vi "[ex ce] Eval y=f(x1,x2).vi"() -> ()   [LabVIEW 2021]
doc: "CE-Math example.\n\n::: CalcExpress Toolkit :::\nCopyright (c) 2000-2026 Konstantin Shifershteyn. All rights reserved."
uses:
  ce exmpl - 2D difference info.ctl
  <vilib>/gmath/NI_Gmath.lvlib
panel:
  out "max relative difference":T1 {"relative difference, %" format="%#.6g"; "absolute difference" format="%#.6g"}
  out "max absolute difference":T1 {"relative difference, %" format="%#.6g"; "absolute difference" format="%#.6g"}
  out "speed ratio":dbl format="%.3f"
  out "GM ticks":u32 caption="ms"
  out "CE ticks":u32 caption="ms"
  out "CE Graph":dbl[][](graph) caption="CalcExpress"
  in  "number of grid points for both variables":u32=100 min=10 max=500
  in  "parameters":cluster{"name":string, "value":dbl}[](array[cluster])=[{"name"="a", "value"=4.0}, {"name"="b", "value"=2.0}] {"value" format="%.2f"}
  in  "formula info":T2={"formula"="a*sinc(x1)-cos(b*x2+pi(1/2))", "variable 1"="x1", "variable 2"="x2"}
  in  "End":cluster{"x1":dbl, "x2":dbl}={"x1"=3.0, "x2"=3.0} {"x2" format="%.2f"; "x1" format="%.2f"}
  in  "Start":cluster{"x1":dbl, "x2":dbl}={"x1"=-3.0, "x2"=-3.0} {"x2" format="%.2f"; "x1" format="%.2f"}
  out "GM Graph":dbl[][](graph) caption="G Math"
  # "NOTE    CalcExpress uses (^) operator to perform bitwise-XOR operation but not power operation.\nYou have to use pow(x,y) function to compute the value of x raised to the y power in CalcExpress."
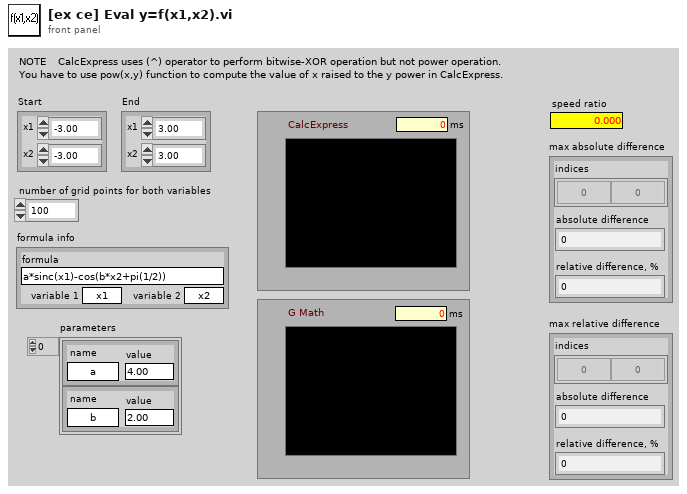
[diagram p1: front panel]
types:
  T1 = typedef "ce exmpl - 2D difference info.ctl" = cluster{"indices":i32[], "absolute difference":dbl, "relative difference, %":dbl}
  T2 = cluster{"formula":string, "variable 1":string, "variable 2":string}
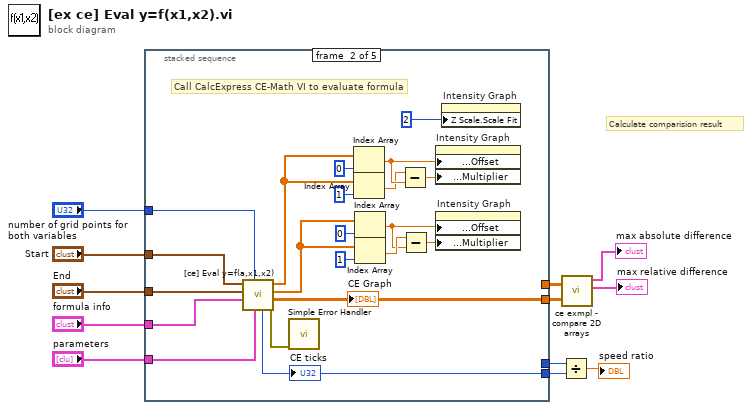
[diagram p0: block diagram]
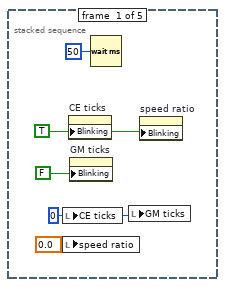
[diagram p2: hidden frame]
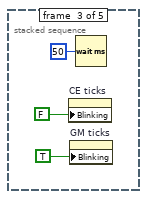
[diagram p3: hidden frame]
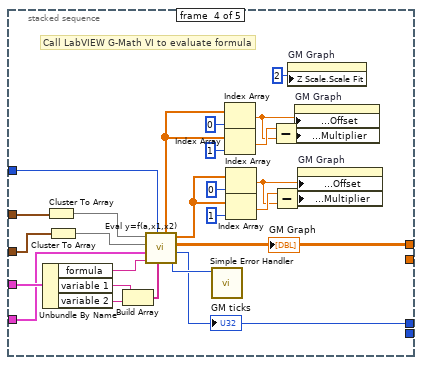
[diagram p4: hidden frame]
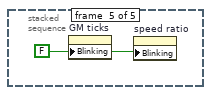
[diagram p5: hidden frame]
diagram:
  # "Calculate comparision result"
  n1 = stacked-sequence {
    tunnel: "Start" -> [_ w34 _ w52 _]
    tunnel: "End" -> [_ w33 _ w51 _]
    tunnel: "formula info" -> [_ w32 _ w50 _]
    tunnel: "parameters" -> [_ w31 _ w49 _]
    tunnel: "number of grid points for both variables" -> [_ w30 _ w53 _]
    tunnel: [_ w29 _ _ _] -> w7
    tunnel: [_ _ _ w48 _] -> w6
    tunnel: [_ w35 _ _ _] -> w5
    tunnel: [_ _ _ w42 _] -> w3
    frame #0 {
      w14 = u32 0 ("CE ticks")
      w16 = TRUE ("Write Attribute")
      n2 = local write "CE ticks"(w14) -> ()
      n3 = local write "speed ratio"(0.0 ("speed ratio")) -> ()
      n4 = property on="CE ticks" class="DigNum (strict)"("Blinking"=w16) -> ()  [unwired: 2 in, 2 out]
      n5 = property on="GM ticks" class="DigNum (strict)"("Blinking"=FALSE ("Write Attribute")) -> ()  [unwired: 2 in, 2 out]
      n6 = Wait (ms)(milliseconds to wait=u32 50) -> ()  [unwired: 1 out]
      n7 = local write "GM ticks"(w14) -> ()
      n8 = property on="speed ratio" class="DigNum (strict)"("Blinking"=w16) -> ()  [unwired: 2 in, 2 out]
    }
    frame #1 {
      # "Call CalcExpress CE-Math VI to evaluate formula"
      n9 = call "[ce] Eval y=f(a,x1,x2).vi"("parameters"=w31, "# points"=w30, "formula info"=w32, "End"=w33, "Start"=w34) -> ("error out"=w38:errorcluster, "Y Values"=w29:dbl[][], "X2  Values"=w36:dbl[], "X1 Values"=w37:dbl[], "ticks"=w35:u32)  [unwired: 2 in]
      "CE Graph" <- w29
      "CE ticks" <- w35
      n10 = call <vilib>:"Simple Error Handler.vi"("error in (no error)"=w38) -> ()  [unwired: 4 in, 5 out]
      n11 = Index Array(array=w37, index=0 ("Index")) -> (element=w28:dbl)
      n12 = Index Array(array=w37, index=1 ("Index")) -> (element=w26:dbl)
      n13 = Index Array(array=w36, index=0 ("Index")) -> (element=w19:dbl)
      n14 = Index Array(array=w36, index=1 ("Index")) -> (element=w21:dbl)
      n15 = Subtract(x=w26, y=w28) -> (x-y=w27:dbl)
      n16 = Subtract(x=w21, y=w19) -> (x-y=w20:dbl)
      n17 = property on="Intensity Graph" class="IntGraph (strict)"("X Scale.Offset and Multiplier:Offset"=w28, "X Scale.Offset and Multiplier:Multiplier"=w27) -> ()  [unwired: 2 in, 2 out]
      n18 = property on="Intensity Graph" class="IntGraph (strict)"("Y Scale.Offset and Multiplier:Offset"=w19, "Y Scale.Offset and Multiplier:Multiplier"=w20) -> ()  [unwired: 2 in, 2 out]
      n19 = property on="Intensity Graph" class="IntGraph (strict)"("Z Scale.Scale Fit"=u8 2 ("Write Attribute")) -> ()  [unwired: 2 in, 2 out]
    }
    frame #2 {
      n20 = property on="CE ticks" class="DigNum (strict)"("Blinking"=FALSE ("Write Attribute")) -> ()  [unwired: 2 in, 2 out]
      n21 = property on="GM ticks" class="DigNum (strict)"("Blinking"=TRUE ("Write Attribute")) -> ()  [unwired: 2 in, 2 out]
      n22 = Wait (ms)(milliseconds to wait=u32 50) -> ()  [unwired: 1 out]
    }
    frame #3 {
      # "Call LabVIEW G-Math VI to evaluate formula"
      n23 = Unbundle By Name(w50) -> ("formula"=w58:string, "variable 1"=w59:string, "variable 2"=w60:string)
      n24 = Cluster To Array(cluster=w52) -> (array=w56:dbl[])
      n25 = Cluster To Array(cluster=w51) -> (array=w57:dbl[])
      n26 = Build Array(w59, w60) -> (w61:string[])
      n27 = call <vilib>:"Eval y=f(a,x1,x2).vi"("Variables"=w61, "number of points"=w53, "formula"=w58, "Parameters"=w49, "End"=w57, "Start"=w56) -> ("error"=w62:i32, "ticks"=w42:u32, "Y Values"=w48:dbl[][], "X2 Values"=w54:dbl[], "X1 Values"=w55:dbl[])
      "GM Graph" <- w48
      "GM ticks" <- w42
      n28 = call <vilib>:"Simple Error Handler.vi"("error code (no error:0)"=w62) -> ()  [unwired: 4 in, 5 out]
      n29 = Index Array(array=w55, index=0 ("Index")) -> (element=w44:dbl)
      n30 = Index Array(array=w55, index=1 ("Index")) -> (element=w68:dbl)
      n31 = Index Array(array=w54, index=0 ("Index")) -> (element=w47:dbl)
      n32 = Index Array(array=w54, index=1 ("Index")) -> (element=w63:dbl)
      n33 = Subtract(x=w68, y=w44) -> (x-y=w45:dbl)
      n34 = Subtract(x=w63, y=w47) -> (x-y=w46:dbl)
      n35 = property on="GM Graph" class="IntGraph (strict)"("Z Scale.Scale Fit"=u8 2 ("Write Attribute")) -> ()  [unwired: 2 in, 2 out]
      n36 = property on="GM Graph" class="IntGraph (strict)"("X Scale.Offset and Multiplier:Offset"=w44, "X Scale.Offset and Multiplier:Multiplier"=w45) -> ()  [unwired: 2 in, 2 out]
      n37 = property on="GM Graph" class="IntGraph (strict)"("Y Scale.Offset and Multiplier:Offset"=w47, "Y Scale.Offset and Multiplier:Multiplier"=w46) -> ()  [unwired: 2 in, 2 out]
    }
    frame #4 {
      w69 = FALSE ("Write Attribute")
      n38 = property on="GM ticks" class="DigNum (strict)"("Blinking"=w69) -> ()  [unwired: 2 in, 2 out]
      n39 = property on="speed ratio" class="DigNum (strict)"("Blinking"=w69) -> ()  [unwired: 2 in, 2 out]
    }
  }
  n40 = Divide(x=w3, y=w5) -> (x/y=→"speed ratio":dbl)
  n41 = call "ce exmpl - compare 2D arrays.vi"("array for checking"=w7, "standard array"=w6) -> ("max relative difference"=→"max relative difference":T1, "max absolute difference"=→"max absolute difference":T1)  [unwired: 1 in, 2 out]
